vi "ISO8601 String to Timestamp.vi"(9 "Strict ISO? (T)":bool=TRUE, 11 "ISO8601 String":string) -> (1 "valid?":bool, 2 "ISO Format":T1, 3 "Timestamp":timestamp)   [LabVIEW 2013]
uses:
  ISO8601 Date Formats.ctl
  <vilib>/Utility/miscctls.llb/LVDateTimeRec.ctl
  Timestamp to ISO8601 Day.vi
  isLeapYear (integer).vi
  <vilib>/regexp/Match Regular Expression.xnode
  DateTime.ISO8601.lvclass
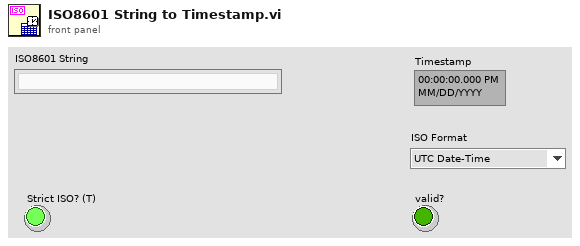
[diagram p1: front panel]
types:
  T1 = typedef "ISO8601 Date Formats.ctl" = enum16{"UTC Date-Time", "ISO Time", "Date", "Calendar Month", "Week", "Week-Day", "Month-Day", "Ordinal Date"}
  T2 = typedef "LVDateTimeRec.ctl" = cluster{"fractional second":dbl, "second":i32, "minute":i32, "hour":i32, "day of month":i32, "month":i32, "year":i32, "day of week":i32, "day of year":i32, "DST":i32}
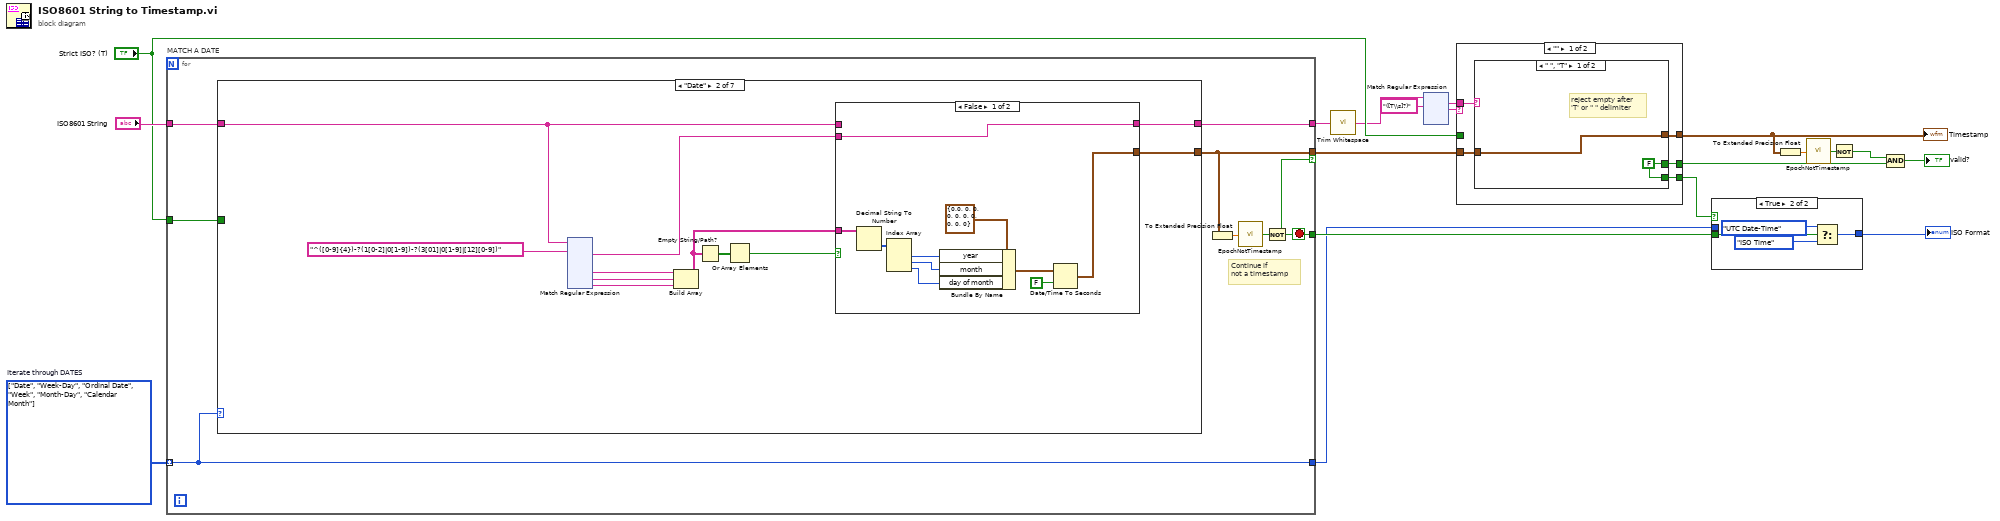
[diagram p0: block diagram]
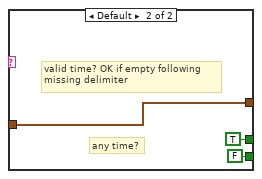
[diagram p2: hidden frame]
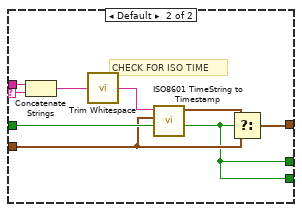
[diagram p3: hidden frame]
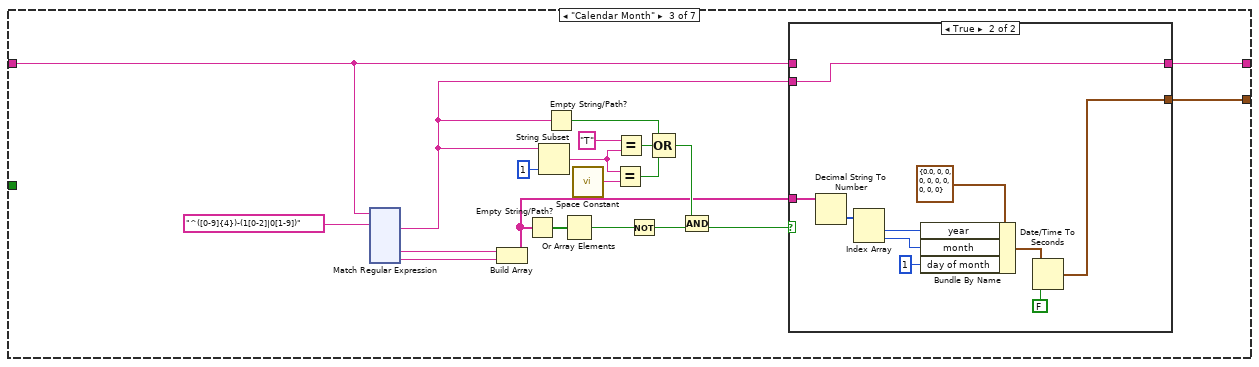
[diagram p6: hidden frame]
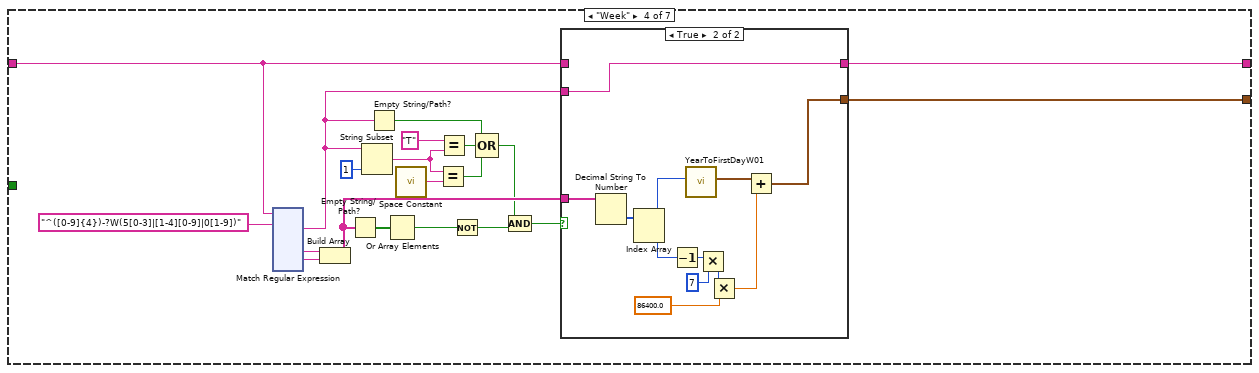
[diagram p8: hidden frame]
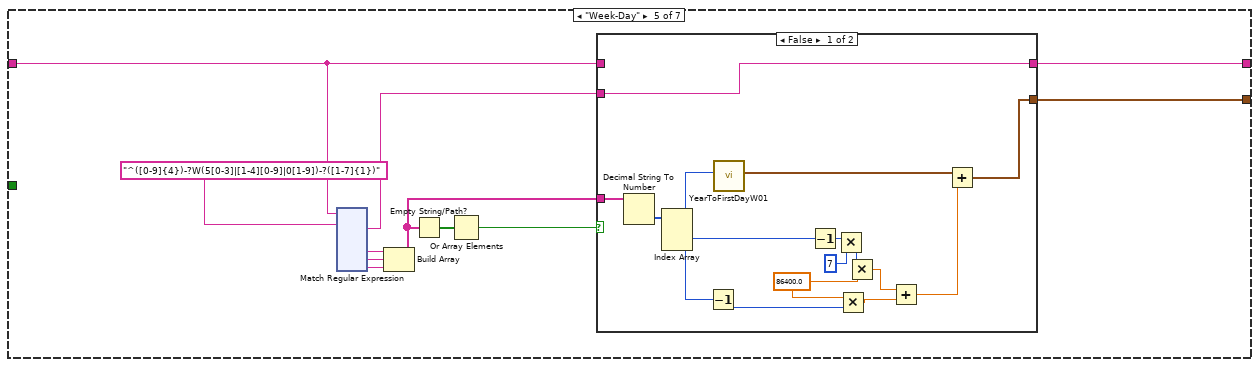
[diagram p10: hidden frame]
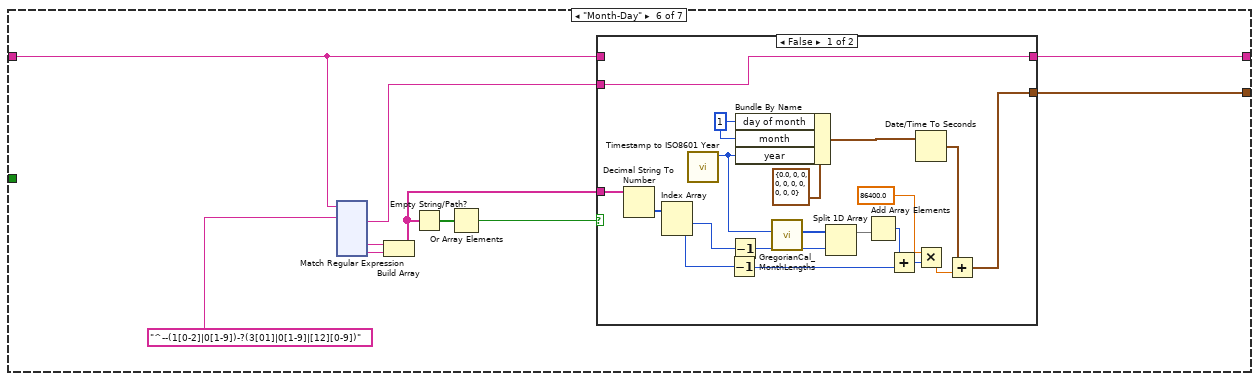
[diagram p12: hidden frame]
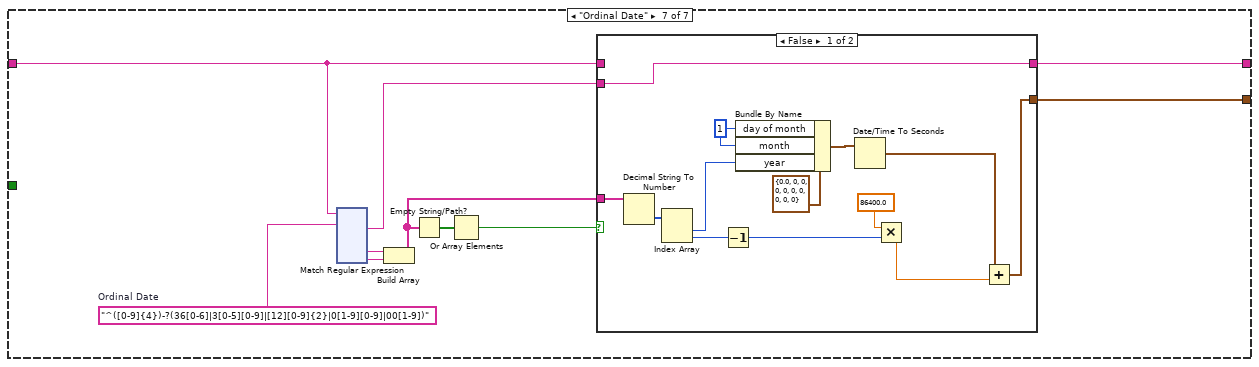
[diagram p14: hidden frame]
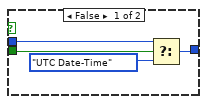
[diagram p16: hidden frame]
diagram:
  w19 = T1[] [enum."Date", enum."Week-Day", enum."Ordinal Date", enum."Week", enum."Month-Day", enum."Calendar Month"] items=["UTC Date-Time", "ISO Time", "Date", "Calendar Month", "Week", "Week-Day", "Month-Day", "Ordinal Date"]  # Iterate through DATES
  n1 = for "MATCH A DATE" {
    tunnel: "ISO8601 String" -> [w27]
    tunnel: [w20] -> w13
    tunnel: [w24] -> w11
    tunnel: w19 -> [w24] mode=indexing
    tunnel: "Strict ISO? (T)" -> [w23]
    tunnel: [w22] -> w18
    tunnel: [w21] -> w14 if=w20
    stop <- w20 stop-if-true
    # "Continue if\nnot a timestamp"
    n2 = case shown="\"Date\"" w24 {
      tunnel: w27 -> [w28 w29 w169 w329 w468 w614 w761]
      tunnel: w23 -> [_ _ _ _ _ _ _]
      tunnel: [w28 w31 w187 w330 w469 w615 w763] -> w22
      tunnel: [_ w32 w188 w331 w471 w617 w764] -> w21
      frame Default {
        # "We process only DATES in this loop."
      }
      frame "Date" {
        n3 = xnode "Match Regular Expression"("input string"=w29, "regular expression"="^([0-9]{4})-?(1[0-2]|0[1-9])-?(3[01]|0[1-9]|[12][0-9])") -> ("after match"=w30:string, "submatch 1"=w39:string, "submatch 2"=w38:string, "submatch 3"=w37:string)  [unwired: 4 in, 4 out]
        n4 = Build Array(w39, w38, w37) -> (w33:string[])
        n5 = Empty String/Path?(string/path=w33) -> (empty?=w36:bool[])
        n6 = Or Array Elements(Boolean array=w36) -> (logical OR=w35:bool)
        n7 = case shown="False" w35 {
          tunnel: w33 -> [w166 _]
          tunnel: [w160 _] -> w32
          tunnel: [w159 w168] -> w31
          tunnel: w30 -> [w159 _]
          tunnel: w29 -> [_ w168]
          frame False {
            n8 = Decimal String To Number(string=w166) -> (number=w167:i32[])  [unwired: 2 in, 1 out]
            n9 = Index Array(array=w167) -> (element #1=w165:i32, element #2=w164:i32, element #3=w163:i32)  [unwired: 3 in]
            n10 = Bundle By Name(cluster=T2 {"fractional second"=0.0, "second"=0, "minute"=0, "hour"=0, "day of month"=0, "month"=0, "year"=0, "day of week"=0, "day of year"=0, "DST"=0} ("date time rec"), "year"=w165, "month"=w164, "day of month"=w163) -> (w162:T2)
            n11 = Date/Time To Seconds(1:FALSE ("is UTC (F)"), 2:w162) -> (0:w160:timestamp)
          }
          frame True {
          }
        }
      }
      frame "Calendar Month" {
        n12 = xnode "Match Regular Expression"("input string"=w169, "regular expression"="^([0-9]{4})-(1[0-2]|0[1-9])") -> ("after match"=w172:string, "submatch 1"=w173:string, "submatch 2"=w174:string)  [unwired: 4 in, 4 out]
        n13 = Build Array(w173, w174) -> (w171:string[])
        n14 = Empty String/Path?(string/path=w171) -> (empty?=w175:bool[])
        n15 = String Subset(string=w172, length (rest)=1 ("length (rest)")) -> (substring=w180:string)  [unwired: 1 in]
        n16 = Empty String/Path?(string/path=w172) -> (empty?=w176:bool)
        n17 = Or Array Elements(Boolean array=w175) -> (logical OR=w184:bool)
        n18 = call <vilib>:"Space Constant.vi"() -> ("String"=w182:string)
        n19 = Equal?(x=w180, y=w182) -> (x = y?=w181:bool)
        n20 = Equal?(x="T", y=w180) -> (x = y?=w179:bool)
        n21 = Not(x=w184) -> (.not. x?=w185:bool)
        n22 = Compound Arithmetic op=OR(w176, w179, w181) -> (w183:bool)
        n23 = Compound Arithmetic op=AND(w183, w185) -> (w170:bool)
        n24 = case shown="True" w170 {
          tunnel: w171 -> [_ w313]
          tunnel: [_ w308] -> w188
          tunnel: w169 -> [w306 _]
          tunnel: [w306 w307] -> w187
          tunnel: w172 -> [_ w307]
          frame False {
          }
          frame True {
            n25 = Decimal String To Number(string=w313) -> (number=w315:i32[])  [unwired: 2 in, 1 out]
            n26 = Index Array(array=w315) -> (element #1=w312:i32, element #2=w311:i32)  [unwired: 2 in]
            n27 = Bundle By Name(cluster=T2 {"fractional second"=0.0, "second"=0, "minute"=0, "hour"=0, "day of month"=0, "month"=0, "year"=0, "day of week"=0, "day of year"=0, "DST"=0} ("date time rec"), "year"=w312, "month"=w311, "day of month"=1) -> (w310:T2)
            n28 = Date/Time To Seconds(1:FALSE ("is UTC (F)"), 2:w310) -> (0:w308:timestamp)
          }
        }
      }
      frame "Week" {
        n29 = xnode "Match Regular Expression"("input string"=w329, "regular expression"="^([0-9]{4})-?W(5[0-3]|[1-4][0-9]|0[1-9])") -> ("after match"=w327:string, "submatch 1"=w336:string, "submatch 2"=w335:string)  [unwired: 4 in, 5 out]
        n30 = Build Array(w336, w335) -> (w332:string[])
        n31 = Empty String/Path?(string/path=w332) -> (empty?=w334:bool[])
        n32 = String Subset(string=w327, length (rest)=1 ("length (rest)")) -> (substring=w323:string)  [unwired: 1 in]
        n33 = Empty String/Path?(string/path=w327) -> (empty?=w328:bool)
        n34 = Or Array Elements(Boolean array=w334) -> (logical OR=w319:bool)
        n35 = call <vilib>:"Space Constant.vi"() -> ("String"=w321:string)
        n36 = Equal?(x=w323, y=w321) -> (x = y?=w322:bool)
        n37 = Equal?(x="T", y=w323) -> (x = y?=w324:bool)
        n38 = Not(x=w319) -> (.not. x?=w318:bool)
        n39 = Compound Arithmetic op=OR(w328, w324, w322) -> (w320:bool)
        n40 = Compound Arithmetic op=AND(w320, w318) -> (w317:bool)
        n41 = case shown="True" w317 {
          tunnel: w332 -> [_ w466]
          tunnel: [_ w457] -> w331
          tunnel: [w455 w456] -> w330
          tunnel: w327 -> [_ w456]
          tunnel: w329 -> [w455 _]
          frame False {
          }
          frame True {
            n42 = Decimal String To Number(string=w466) -> (number=w467:i32[])  [unwired: 2 in, 1 out]
            n43 = Index Array(array=w467) -> (element #1=w465:i32, element #2=w464:i32)  [unwired: 2 in]
            n44 = Decrement(x=w464) -> (x-1=w463:i32)
            n45 = call "YearToFirstDayW01.vi"("year"=w465) -> ("First Day of W01"=w459:timestamp)  [unwired: 10 in]
            n46 = Multiply(x=w463, y=7) -> (x*y=w462:i32)
            n47 = Multiply(x=w462, y=86400.0) -> (x*y=w458:dbl)
            n48 = Add(x=w459, y=w458) -> (x+y=w457:timestamp)
          }
        }
      }
      frame "Week-Day" {
        n49 = xnode "Match Regular Expression"("input string"=w468, "regular expression"="^([0-9]{4})-?W(5[0-3]|[1-4][0-9]|0[1-9])-?([1-7]{1})") -> ("after match"=w470:string, "submatch 1"=w478:string, "submatch 2"=w477:string, "submatch 3"=w473:string)  [unwired: 4 in, 4 out]
        n50 = Build Array(w478, w477, w473) -> (w474:string[])
        n51 = Empty String/Path?(string/path=w474) -> (empty?=w476:bool[])
        n52 = Or Array Elements(Boolean array=w476) -> (logical OR=w475:bool)
        n53 = case shown="False" w475 {
          tunnel: w474 -> [w611 _]
          tunnel: [w598 _] -> w471
          tunnel: [w597 w613] -> w469
          tunnel: w470 -> [w597 _]
          tunnel: w468 -> [_ w613]
          frame False {
            w601 = 86400.0
            n54 = Decimal String To Number(string=w611) -> (number=w612:i32[])  [unwired: 2 in, 1 out]
            n55 = Index Array(array=w612) -> (element #1=w610:i32, element #2=w609:i32, element #3=w602:i32)  [unwired: 3 in]
            n56 = Decrement(x=w602) -> (x-1=w600:i32)
            n57 = call "YearToFirstDayW01.vi"("year"=w610) -> ("First Day of W01"=w605:timestamp)  [unwired: 10 in]
            n58 = Decrement(x=w609) -> (x-1=w608:i32)
            n59 = Multiply(x=w608, y=7) -> (x*y=w607:i32)
            n60 = Multiply(x=w601, y=w600) -> (x*y=w599:dbl)
            n61 = Multiply(x=w607, y=w601) -> (x*y=w604:dbl)
            n62 = Add(x=w604, y=w599) -> (x+y=w603:dbl)
            n63 = Add(x=w605, y=w603) -> (x+y=w598:timestamp)
          }
          frame True {
          }
        }
      }
      frame "Month-Day" {
        n64 = xnode "Match Regular Expression"("input string"=w614, "regular expression"="^--(1[0-2]|0[1-9])-?(3[01]|0[1-9]|[12][0-9])") -> ("after match"=w616:string, "submatch 1"=w623:string, "submatch 2"=w622:string)  [unwired: 4 in, 4 out]
        n65 = Build Array(w623, w622) -> (w619:string[])
        n66 = Empty String/Path?(string/path=w619) -> (empty?=w621:bool[])
        n67 = Or Array Elements(Boolean array=w621) -> (logical OR=w620:bool)
        n68 = case shown="False" w620 {
          tunnel: w619 -> [w758 _]
          tunnel: [w742 _] -> w617
          tunnel: w616 -> [w741 _]
          tunnel: [w741 w760] -> w615
          tunnel: w614 -> [_ w760]
          frame False {
            w754 = 1 ("day of month")
            n69 = Decimal String To Number(string=w758) -> (number=w759:i32[])  [unwired: 2 in, 1 out]
            n70 = Index Array(array=w759) -> (element #1=w749:i32, element #2=w757:i32)  [unwired: 2 in]
            n71 = call "Timestamp to ISO8601 Year.vi"() -> ("year"=w751:i32)  [unwired: 10 in, 1 out]
            n72 = Decrement(x=w757) -> (x-1=w745:i32)
            n73 = Decrement(x=w749) -> (x-1=w748:i32)
            n74 = Bundle By Name(cluster=T2 {"fractional second"=0.0, "second"=0, "minute"=0, "hour"=0, "day of month"=0, "month"=0, "year"=0, "day of week"=0, "day of year"=0, "DST"=0} ("date time rec"), "day of month"=w754, "month"=w754, "year"=w751) -> (w755:T2)
            n75 = call "GregorianCal_MonthLengths.vi"("Year (0: this year)"=w751) -> ("Month Lengths"=w750:i32[])  [unwired: 10 in]
            n76 = Split 1D Array(array=w750, index=w748) -> (first subarray=w747:i32[])  [unwired: 1 out]
            n77 = Add Array Elements(numeric array=w747) -> (sum=w746:i32)
            n78 = Add(x=w746, y=w745) -> (x+y=w744:i32)
            n79 = Date/Time To Seconds(2:w755) -> (0:w752:timestamp)  [unwired: 1 in]
            n80 = Multiply(x=86400.0, y=w744) -> (x*y=w743:dbl)
            n81 = Add(x=w752, y=w743) -> (x+y=w742:timestamp)
          }
          frame True {
          }
        }
      }
      frame "Ordinal Date" {
        w765 = "^([0-9]{4})-?(36[0-6]|3[0-5][0-9]|[12][0-9]{2}|0[1-9][0-9]|00[1-9])"  # Ordinal Date
        n82 = xnode "Match Regular Expression"("input string"=w761, "regular expression"=w765) -> ("after match"=w762:string, "submatch 1"=w770:string, "submatch 2"=w769:string)  [unwired: 4 in, 4 out]
        n83 = Build Array(w770, w769) -> (w766:string[])
        n84 = Empty String/Path?(string/path=w766) -> (empty?=w768:bool[])
        n85 = Or Array Elements(Boolean array=w768) -> (logical OR=w767:bool)
        n86 = case shown="False" w767 {
          tunnel: w766 -> [w899 _]
          tunnel: [w889 _] -> w764
          tunnel: [w888 w901] -> w763
          tunnel: w762 -> [w888 _]
          tunnel: w761 -> [_ w901]
          frame False {
            w895 = 1 ("day of month")
            n87 = Decimal String To Number(string=w899) -> (number=w900:i32[])  [unwired: 2 in, 1 out]
            n88 = Index Array(array=w900) -> (element #1=w892:i32, element #2=w898:i32)  [unwired: 2 in]
            n89 = Decrement(x=w898) -> (x-1=w891:i32)
            n90 = Bundle By Name(cluster=T2 {"fractional second"=0.0, "second"=0, "minute"=0, "hour"=0, "day of month"=0, "month"=0, "year"=0, "day of week"=0, "day of year"=0, "DST"=0} ("date time rec"), "day of month"=w895, "month"=w895, "year"=w892) -> (w896:T2)
            n91 = Date/Time To Seconds(2:w896) -> (0:w890:timestamp)  [unwired: 1 in]
            n92 = Multiply(x=86400.0, y=w891) -> (x*y=w893:dbl)
            n93 = Add(x=w890, y=w893) -> (x+y=w889:timestamp)
          }
          frame True {
          }
        }
      }
    }
    n94 = To Extended Precision Float(1:w21) -> (0:w26:ext)
    n95 = call "EpochNotTimestamp.vi"("Epoch Time"=w26) -> ("Not a Timestamp?"=w25:bool)  [unwired: 8 in]
    n96 = Not(x=w25) -> (.not. x?=w20:bool)
  }
  n97 = call <vilib>:"Trim Whitespace.vi"("string"=w18) -> ("trimmed string"=w5:string)  [unwired: 1 in]
  n98 = xnode "Match Regular Expression"("input string"=w5, "regular expression"="([T\\s]?)") -> ("whole match"=w3:string, "after match"=w4:string)  [unwired: 4 in, 3 out]
  n99 = case shown="\"\"" w4 {
    selector: w4 -> [_ w917]
    tunnel: [w903 w920] -> w15
    tunnel: w14 -> [w904 w916]
    tunnel: [w906 w914] -> w2
    tunnel: "Strict ISO? (T)" -> [_ w919]
    tunnel: w3 -> [w905 w918]
    tunnel: [w902 w914] -> w1
    frame "" {
      n100 = case shown="\" \", \"T\"" w905 {
        tunnel: [w907 TRUE ("valid?")] -> w906
        tunnel: w904 -> [w908 w910]
        tunnel: [w908 w910] -> w903
        tunnel: [w907 FALSE ("valid?")] -> w902
        frame " ", "T" {
          w907 = FALSE ("valid?")
          # "reject empty after\n'T' or \" \" delimiter"
        }
        frame Default {
          # "any time?"
          # "valid time? OK if empty following\nmissing delimiter"
        }
      }
    }
    frame Default {
      # "CHECK FOR ISO TIME"
      n101 = Concatenate Strings(w918, w917) -> (w913:string)
      n102 = call <vilib>:"Trim Whitespace.vi"("string"=w913) -> ("trimmed string"=w912:string)  [unwired: 1 in]
      n103 = call "ISO8601 TimeString to Timestamp.vi"("Strict ISO? (T)"=w919, "Date (today)"=w916, "ISO8601 Time String"=w912) -> ("valid?"=w914:bool, "Timestamp"=w915:timestamp)  [unwired: 7 in]
      n104 = Select(t=w915, s=w914, f=w916) -> (s? t:f=w920:timestamp)
    }
  }
  "Timestamp" <- w15
  n105 = case shown="True" w1 {
    tunnel: w13 -> [w924 w926]
    tunnel: [w922 w925] -> w12
    tunnel: w11 -> [w921 _]
    frame False {
      n106 = Select(t=w921, s=w924, f=ISO8601_Date_Formats."UTC Date-Time" ("ISO Format")) -> (s? t:f=w922:T1)
    }
    frame True {
      n107 = Select(t=ISO8601_Date_Formats."UTC Date-Time" ("ISO Format"), s=w926, f=ISO8601_Date_Formats."ISO Time" ("ISO Format")) -> (s? t:f=w925:T1)
    }
  }
  "ISO Format" <- w12
  n108 = To Extended Precision Float(1:w15) -> (0:w17:ext)
  n109 = call "EpochNotTimestamp.vi"("Epoch Time"=w17) -> ("Not a Timestamp?"=w16:bool)  [unwired: 8 in]
  n110 = Not(x=w16) -> (.not. x?=w9:bool)
  n111 = Compound Arithmetic op=AND(w9, w2) -> (→"valid?":bool)
